vi "GDSAPI_CreateMethods2.vi"(6 "PropertyMethodType":T1, 8 "error in (no error)":errorcluster, 10 "Methods":T2[](array[typedef]), 11 "ClassPath(*.lvclass)":path) -> (0 "error out":errorcluster, 3 "MethodsCreated":path[](array[path]))   [LabVIEW 2020]
doc: "This VI creates Methods in a class."
uses:
  ClassProviders/Common/String/GDSString_MethodDescriptionType.ctl
  ClassProviders/Common/CommonVIs/CommonVIs_AttributeType.ctl
  ClassProviders/Common/CommonVIs/CommonVIs_AttributeDataType.ctl
  ClassProviders/Common/String/GDSString_AccessScopeModifierType.ctl
  ClassProviders/Common/String/GDSString_ModifierType.ctl
  ClassProviders/Common/CommonVIs/CommonVIs_PropertyType.ctl
  GDSAPI_SubVIs/GDSAPI_PropertyMethodType.ctl
  GDSAPI_SubVIs/GDSAPI_MethodType.ctl
  ClassProviders/Provider_BaseClassInterface/CreateMethodData.ctl
  ClassProviders/Provider_EndevoGOOP300/GOOP300_SubVIs/GOOP300_MethodScopeType.ctl
  ClassProviders/Provider_LvNativeClass/ClassWriterNative_class/IconDetails.ctl
  ClassProviders/Provider_LvNativeClass/ClassWriterNative_class/IconSize.ctl
  ClassProviders/Provider_LvNativeClass/ClassWriterNative_class/ClassWriterNative.lvclass
  ClassProviders/Provider_BaseClassInterface/ClassWriter_class/ClassWriter.lvclass
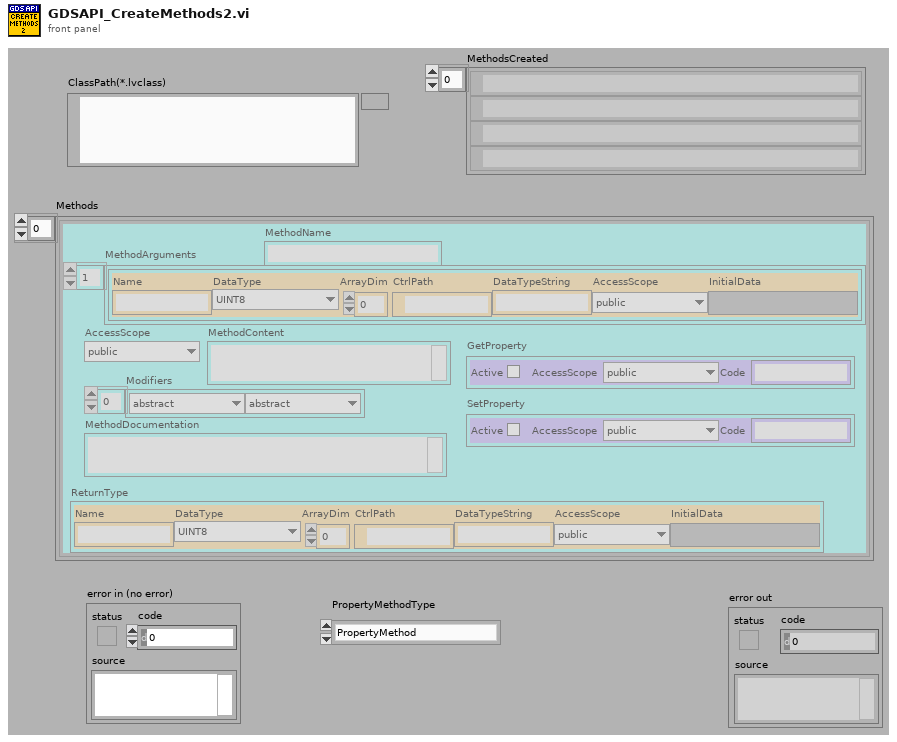
[diagram p1: front panel]
types:
  T1 = typedef "GDSAPI_PropertyMethodType.ctl" = enum16{"PropertyMethod", "PropertyNode"}
  T2 = typedef "GDSString_MethodDescriptionType.ctl" = cluster{"ReturnType":T3, "MethodName":string, "AccessScope":T5, "Modifiers":T6[], "MethodDocumentation":string, "MethodContent":string, "MethodArguments":T3[], "GetProperty":T7, "SetProperty":T7}
  T3 = typedef "CommonVIs_AttributeType.ctl" = cluster{"Name":string, "DataType":T4, "ArrayDim":i32, "CtrlPath":path, "DataTypeString":string, "AccessScope":T5, "InitialData":variant}
  T4 = typedef "CommonVIs_AttributeDataType.ctl" = enum16{"UINT8", "INT8", "UINT16", "INT16", "UINT32", "INT32", "UINT64", "INT64", "SGL", "DBL", "EXT", "CSG", "CDB", "CXT", "TimeStamp", "STRING", "PATH", "BOOL", "ENUM", "RefNum", "VIRefNum", "LabVIEW Class", "Cluster", "Variant", "TypeDef", "Waveform", "LabVIEW Object", "Other", "void", "Set", "Map"}
  T5 = typedef "GDSString_AccessScopeModifierType.ctl" = enum16{"public", "private", "protected", "internal"}
  T6 = typedef "GDSString_ModifierType.ctl" = enum16{"abstract", "static", "final", "synchronized", "strictfp", "async", "const", "event", "extern", "new", "native ", "override", "partial", "readonly", "sealed", "unsafe", "virtual", "volatile"}
  T7 = typedef "CommonVIs_PropertyType.ctl" = cluster{"Active":bool, "AccessScope":T5, "Code":string}
  T8 = typedef "GDSAPI_MethodType.ctl" = enum16{"Read Attribute", "Write Attribute", "Read & Write Attribute", "None Modifying Method", "Get Property", "Set Property", "Read Property", "Write Property", "Static Method", "Interface Method"}
  T9 = cluster{"AttributeNames":string[], "PropertyNode":bool, "FolderNames":string[]}
  T10 = typedef "ClassWriter.lvclass/CreateMethodData.ctl" = cluster{"MethodName":string, "RelativeMethodPath":path, "MethodDescription":string, "Scope/Visibility":T11, "MethodTemplateName":string, "IconOut":u8[][], "RelativeProjectClassPath":string, "OpenViAfterCreation":bool, "DynamicDispatchVi":bool, "ExtraCreateParameters":variant, "MustOverride":bool, "MustCallParent":bool, "IconDetails":T12, "AF-Option":variant, "TemplatePath":path}
  T11 = typedef "GOOP300_MethodScopeType.ctl" = enum16{"Use Parent Folder Scope", "Public", "Protected", "Private", "Community"}
  T12 = typedef "ClassWriterNative.lvclass/IconDetails.ctl" = cluster{"IconSize":T13, "ImageRows(32)":i32, "ConnectorPaneHeight":i32[]}
  T13 = typedef "ClassWriterNative.lvclass/IconSize.ctl" = enum16{"Full", "1 c-term high", "2 c-term high", "3 c-term high"}
  T14 = typedef "GDSLvCLass_ClassSettingsType.ctl" = cluster{"ClassProviderName":string, "ClassTemplateUsed":string, "ClassTemplateVersion":string, "ClassDescription":string, "PlugIns":T15[], "ConnectorPanePattern":string}
  T15 = typedef "GDSLvClass_PlugIn.ctl" = cluster{"Type":T16, "ID":string, "Version":string, "Path":path, "Name":string, "Data":variant}
  T16 = typedef "GDSLvClass_PlugInTypes.ctl" = enum16{"DesignPattern", "MethodTypes"}
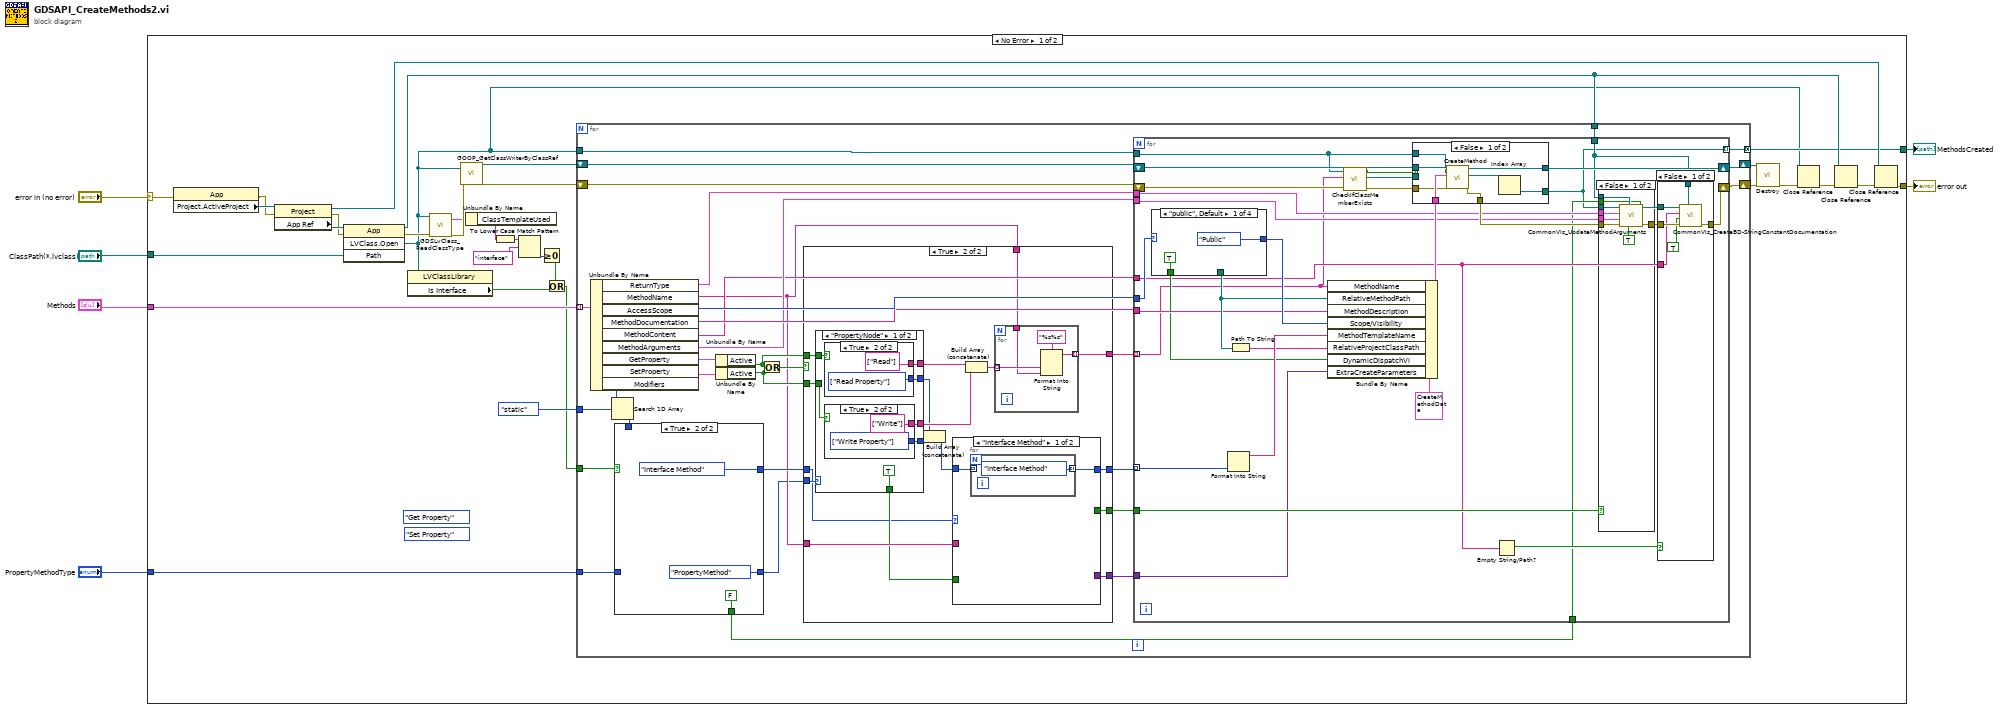
[diagram p0: block diagram]
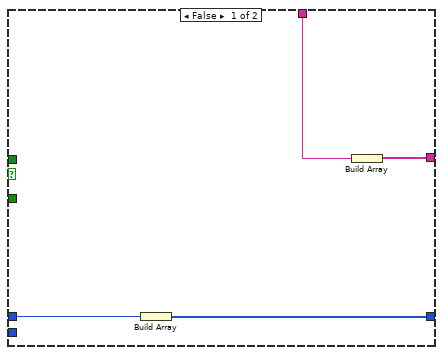
[diagram p2: hidden frame]
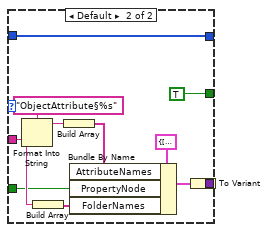
[diagram p3: hidden frame]
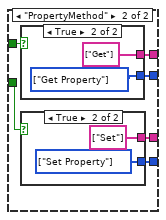
[diagram p6: hidden frame]
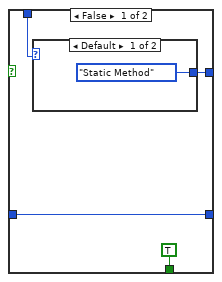
[diagram p9: hidden frame]
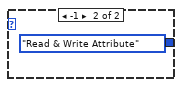
[diagram p10: hidden frame]
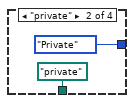
[diagram p14: hidden frame]
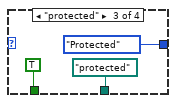
[diagram p15: hidden frame]
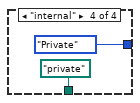
[diagram p16: hidden frame]
diagram:
  n1 = case shown="No Error" "error in (no error)" {
    selector: "error in (no error)" -> [w13 w204]
    tunnel: "ClassPath(*.lvclass)" -> [w37 _]
    tunnel: "Methods" -> [w36 _]
    tunnel: [w24 w204] -> w4
    tunnel: "PropertyMethodType" -> [w16 _]
    tunnel: [w11 _] -> w1
    frame No Error {
      (unwired) GDSAPI_MethodType."Set Property" ("MethodType")
      (unwired) GDSAPI_MethodType."Get Property" ("MethodType")
      n2 = property class="App"(error in=w13) -> (error out=w27:errorcluster, "Project.ActiveProject"=w30:refnum<vi>)  [unwired: 1 in, 1 out]
      n3 = property class="Project"(reference=w30, error in=w27) -> (reference out=w15:refnum<vi>, error out=w28:errorcluster, "App Ref"=w29:refnum<vi>)
      n4 = invoke class="App" method="LVClass.Open"(reference=w29, error in=w28, "Path"=w37) -> (reference out=w14:refnum<vi>, error out=w23:errorcluster, "LVClass.Open"=w10:refnum<vi>)  [unwired: 1 in, 1 out]
      n5 = property class="LVClassLibrary"(reference=w10) -> ("Is Interface"=w8:bool)  [unwired: 1 in, 2 out]
      n6 = call "GDSLvClass_ReadClassType.vi"("Class Refnum In"=w10, "error in (no error)"=w23) -> ("ClassSettings"=w21:T14, "error out"=w22:errorcluster)  [unwired: 15 in, 1 out]
      n7 = call "GOOP_GetClassWriterByClassRef.vi"("LVClassLibrary Refnum"=w10, "error in (no error)"=w22) -> ("ClassWriterNative.lvclass"=w31:refnum<class "ClassWriterNative.lvclass">, "error out"=w32:errorcluster)  [unwired: 16 in]
      n8 = Unbundle By Name(w21) -> ("ClassTemplateUsed"=w20:string)
      n9 = To Lower Case(string=w20) -> (all lower case string=w19:string)
      n10 = Match Pattern(string=w19, regular expression="interface") -> (offset past match=w17:i32)  [unwired: 1 in, 3 out]
      n11 = Greater Or Equal To 0?(x=w17) -> (x >= 0?=w9:bool)
      n12 = Or(x=w9, y=w8) -> (x .or. y?=w7:bool)
      n13 = for {
        tunnel: w10 -> [w66]
        tunnel: w36 -> [w64] mode=indexing
        shift-right: [w61] -> w33
        shift-left: w32 -> [w67]
        shift-right: [w68] -> w34
        shift-left: w31 -> [w65]
        tunnel: w7 -> [w56]
        tunnel: w16 -> [w41]
        tunnel: w14 -> [w48]
        tunnel: GDSString_ModifierType."static" ("element") -> [w44]
        tunnel: [w38] -> w11 mode=concatenating
        n14 = Unbundle By Name(w64) -> ("ReturnType"=w60:T3, "MethodName"=w42:string, "AccessScope"=w63:T5, "MethodDocumentation"=w62:string, "MethodContent"=w47:string, "MethodArguments"=w59:T3[], "GetProperty"=w58:T7, "SetProperty"=w57:T7, "Modifiers"=w45:T6[])
        n15 = Search 1D Array(1D array=w45, element=w44) -> (index of element=w43:i32)  [unwired: 1 in]
        n16 = case shown="True" w56 {
          tunnel: [w132 GDSAPI_MethodType."Interface Method" ("MethodType")] -> w55
          tunnel: w43 -> [w131 _]
          tunnel: w41 -> [w130 _]
          tunnel: [w130 GDSAPI_PropertyMethodType."PropertyMethod" ("PropertyMethodType")] -> w40
          tunnel: [TRUE FALSE] -> w39
          frame False {
            n17 = case shown="Default" w131 {
              tunnel: [GDSAPI_MethodType."Static Method" ("MethodType") GDSAPI_MethodType."Read & Write Attribute" ("MethodType")] -> w132
              frame Default {
              }
              frame -1 {
              }
            }
          }
          frame True {
          }
        }
        n18 = Unbundle By Name(w58) -> ("Active"=w52:bool)
        n19 = Unbundle By Name(w57) -> ("Active"=w51:bool)
        n20 = Or(x=w52, y=w51) -> (x .or. y?=w53:bool)
        n21 = case shown="True" w53 {
          tunnel: w55 -> [w72 w76]
          tunnel: [w71 w88] -> w54
          tunnel: w52 -> [_ w89]
          tunnel: w51 -> [_ w87]
          tunnel: w40 -> [_ w86]
          tunnel: w42 -> [w69 w81]
          tunnel: [_ w85] -> w50
          tunnel: [_ w84] -> w49
          tunnel: w42 -> [_ w83]
          tunnel: [w70 w80] -> w46
          frame False {
            n22 = Build Array(w72) -> (w71:T8[])
            n23 = Build Array(w69) -> (w70:string[])
          }
          frame True {
            n24 = case shown="\"PropertyNode\"" w86 {
              tunnel: w89 -> [w114 w124]
              tunnel: w87 -> [w113 w123]
              tunnel: [w112 w122] -> w74
              tunnel: [w111 w121] -> w75
              tunnel: [TRUE _] -> w82
              tunnel: [w109 w120] -> w78
              tunnel: [w108 w119] -> w77
              frame "PropertyNode" {
                n25 = case shown="True" w114 {
                  tunnel: [_ w118] -> w112
                  tunnel: [_ string[] ["Read"]] -> w109
                  frame False {
                  }
                  frame True {
                    w118 = T8[] [enum."Read Property"] items=["Read Attribute", "Write Attribute", "Read & Write Attribute", "None Modifying Method", "Get Property", "Set Property", "Read Property", "Write Property", "Static Method", "Interface Method"]
                  }
                }
                n26 = case shown="True" w113 {
                  tunnel: [_ w116] -> w111
                  tunnel: [_ string[] ["Write"]] -> w108
                  frame False {
                  }
                  frame True {
                    w116 = T8[] [enum."Write Property"] items=["Read Attribute", "Write Attribute", "Read & Write Attribute", "None Modifying Method", "Get Property", "Set Property", "Read Property", "Write Property", "Static Method", "Interface Method"]
                  }
                }
              }
              frame "PropertyMethod" {
                n27 = case shown="True" w124 {
                  tunnel: [_ w128] -> w122
                  tunnel: [_ string[] ["Get"]] -> w120
                  frame False {
                  }
                  frame True {
                    w128 = T8[] [enum."Get Property"] items=["Read Attribute", "Write Attribute", "Read & Write Attribute", "None Modifying Method", "Get Property", "Set Property", "Read Property", "Write Property", "Static Method", "Interface Method"]
                  }
                }
                n28 = case shown="True" w123 {
                  tunnel: [_ w126] -> w121
                  tunnel: [_ string[] ["Set"]] -> w119
                  frame False {
                  }
                  frame True {
                    w126 = T8[] [enum."Set Property"] items=["Read Attribute", "Write Attribute", "Read & Write Attribute", "None Modifying Method", "Get Property", "Set Property", "Read Property", "Write Property", "Static Method", "Interface Method"]
                  }
                }
              }
            }
            n29 = Build Array (concatenate)(w74, w75) -> (w73:T8[])
            n30 = case shown="\"Interface Method\"" w76 {
              tunnel: [w90 w94] -> w88
              tunnel: w73 -> [w91 w94]
              tunnel: [_ TRUE] -> w85
              tunnel: [_ w97] -> w84
              tunnel: w83 -> [_ w96]
              tunnel: w82 -> [_ w95]
              frame "Interface Method" {
                n31 = for {
                  tunnel: w91 -> [_] mode=indexing
                  tunnel: [GDSAPI_MethodType."Interface Method" ("MethodType")] -> w90 mode=indexing
                }
              }
              frame Default {
                n32 = Format Into String(format string="ObjectAttribute§%s", w96) -> (resulting string=w101:string)  [unwired: 2 in, 1 out]
                n33 = Build Array(w96) -> (w103:string[])
                n34 = Build Array(w101) -> (w102:string[])
                n35 = Bundle By Name(cluster=T9 {"AttributeNames"=[], "PropertyNode"=FALSE, "FolderNames"=[]}, "AttributeNames"=w102, "PropertyNode"=w95, "FolderNames"=w103) -> (w98:T9)
                n36 = To Variant(anything=w98) -> (Variant=w97:variant)
              }
            }
            n37 = Build Array (concatenate)(w78, w77) -> (w79:string[])
            n38 = for {
              tunnel: w79 -> [w107] mode=indexing
              tunnel: w81 -> [w106]
              tunnel: [w105] -> w80 mode=indexing
              n39 = Format Into String(format string="%s%s", w107, w106) -> (resulting string=w105:string)  [unwired: 2 in, 1 out]
            }
          }
        }
        n40 = for {
          tunnel: w66 -> [w143]
          tunnel: w63 -> [w161]
          tunnel: w62 -> [w158]
          tunnel: w54 -> [w153] mode=indexing
          tunnel: w60 -> [w155]
          tunnel: w59 -> [w154]
          shift-right: [w149] -> w61
          shift-left: w67 -> [w145]
          shift-right: [w167] -> w68
          shift-left: w65 -> [w166]
          tunnel: w50 -> [w152]
          tunnel: w49 -> [w151]
          tunnel: w48 -> [w148]
          tunnel: w47 -> [w147]
          tunnel: w46 -> [w140] mode=indexing
          tunnel: w39 -> [w139]
          tunnel: [w138] -> w38 mode=indexing
          n41 = case shown="\"public\", Default" w161 {
            tunnel: [GOOP300_MethodScopeType."Public" ("Scope/Visibility") GOOP300_MethodScopeType."Private" ("Scope/Visibility") GOOP300_MethodScopeType."Protected" ("Scope/Visibility") GOOP300_MethodScopeType."Private" ("Scope/Visibility")] -> w164
            tunnel: [_ path "private" ("RelativeMethodPath") path "protected" ("RelativeMethodPath") path "private" ("RelativeMethodPath")] -> w160
            tunnel: [TRUE _ TRUE _] -> w157
            frame "public", Default {
            }
            frame "private" {
            }
            frame "protected" {
            }
            frame "internal" {
            }
          }
          n42 = Format Into String(w153) -> (resulting string=w162:string)  [unwired: 3 in, 1 out]
          n43 = Path To String(path=w160) -> (string=w159:string)
          n44 = Bundle By Name(cluster=T10 {"MethodName"="", "RelativeMethodPath"=path "", "MethodDescription"="", "Scope/Visibility"=enum."Use Parent Folder Scope", "MethodTemplateName"="", "IconOut"=[], "RelativeProjectClassPath"="", "OpenViAfterCreation"=FALSE, "DynamicDispatchVi"=FALSE, "ExtraCreateParameters"=variant, "MustOverride"=FALSE, "MustCallParent"=FALSE, "IconDetails"={"IconSize"=enum."Full", "ImageRows(32)"=0, "ConnectorPaneHeight"=[]}, "AF-Option"=variant, "TemplatePath"=path ""} ("CreateMethodData"), "MethodName"=w140, "RelativeMethodPath"=w160, "MethodDescription"=w158, "Scope/Visibility"=w164, "MethodTemplateName"=w162, "RelativeProjectClassPath"=w159, "DynamicDispatchVi"=w157, "ExtraCreateParameters"=w151) -> (w163:T10)
          n45 = call "CheckIfClassMemberExists.vi"("error in (no error)"=w145, "MethodName"=w140, "LVClassLibrary in"=w143) -> ("error out"=w144:errorcluster, "Path"=w141:path, "Exists"=w142:bool)  [unwired: 6 in]
          n46 = case shown="False" w142 {
            tunnel: [w175 w178] -> w167
            tunnel: w166 -> [w174 w178]
            tunnel: w163 -> [w173 _]
            tunnel: [w172 w177] -> w156
            tunnel: w144 -> [w171 w177]
            tunnel: w143 -> [w170 _]
            tunnel: [w168 w176] -> w138
            tunnel: w141 -> [_ w176]
            frame False {
              n47 = call-dynamic "CreateMethod.vi"("ClassWriterNative.lvclass"=w174, "ClassItemRefIn"=w170, "CreateMethodData"=w173, "error in (no error)"=w171) -> ("ClassWriterNative.lvclass 2"=w175:refnum<class "ClassWriterNative.lvclass">, "MethodPaths"=w169:path[], "error out"=w172:errorcluster)  [unwired: 12 in, 1 out]
              n48 = Index Array(array=w169) -> (element=w168:path)  [unwired: 1 in]
            }
            frame True {
            }
          }
          n49 = Empty String/Path?(string/path=w147) -> (empty?=w146:bool)
          n50 = case shown="False" w152 {
            tunnel: w138 -> [w193 _]
            tunnel: w156 -> [w192 w194]
            tunnel: [w191 w194] -> w150
            tunnel: w155 -> [w190 _]
            tunnel: w154 -> [w189 _]
            tunnel: w148 -> [w188 _]
            tunnel: w139 -> [w186 _]
            frame False {
              n51 = call "CommonVIs_UpdateMethodArguments.vi"("CleanUpControls(True)"=w186, "Keep Existing Controls And Indicatores connected(False)"=TRUE, "App"=w188, "error in (no error)"=w192, "MethodArguments"=w189, "ReturnType"=w190, "VI Ref/Vi Path"=w193) -> ("error out"=w191:errorcluster)  [unwired: 4 in]
            }
            frame True {
            }
          }
          n52 = case shown="False" w146 {
            tunnel: w150 -> [w184 w185]
            tunnel: [w183 w185] -> w149
            tunnel: w138 -> [w182 _]
            tunnel: w148 -> [w181 _]
            tunnel: w147 -> [w179 _]
            frame False {
              n53 = call "CommonVIs_CreateBD-StringConstantDocumentation.vi"("App"=w181, "error in (no error)"=w184, "Remove extra prefixed spaces on every row but keep indentation"=TRUE ("Remove extar prefixed spaces on every row but keep indentation"), "Documentation"=w179, "VI Ref/Vi Path"=w182) -> ("error out"=w183:errorcluster)  [unwired: 6 in]
            }
            frame True {
            }
          }
        }
      }
      n54 = call-dynamic "Destroy.vi"("ClassWriterNative"=w34, "error in (no error)"=w33) -> ("error out"=w35:errorcluster)  [unwired: 17 in]
      n55 = Close Reference(reference=w10, error in (no error)=w35) -> (error out=w26:errorcluster)
      n56 = Close Reference(reference=w14, error in (no error)=w26) -> (error out=w25:errorcluster)
      n57 = Close Reference(reference=w15, error in (no error)=w25) -> (error out=w24:errorcluster)
    }
    frame Error {
    }
  }
  "error out" <- w4
  "MethodsCreated" <- w1
